vi "RichToFlatcif_can_writer_nixnet_Statistics.vi"(5 "OutputClusterType":T1, 11 "InputCluster":T2) -> (3 "OutputCluster":T1)   [LabVIEW 2021, in "CanWriterNixnet_server.lvlib"]
uses:
  CanWriterNixnet_server.lvlib
  cif_can_writer_nixnet_Statistics.ctl
  cif_can_writer_nixnet_Statistics_Flat.ctl
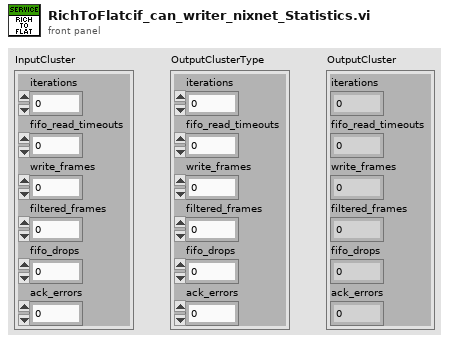
[diagram p1: front panel]
types:
  T1 = typedef "CanWriterNixnet_server.lvlib/cif_can_writer_nixnet_Statistics_Flat.ctl" = cluster{"iterations":u64, "fifo_read_timeouts":u64, "write_frames":u64, "filtered_frames":u64, "fifo_drops":u64, "ack_errors":u64}
  T2 = typedef "CanWriterNixnet_server.lvlib/cif_can_writer_nixnet_Statistics.ctl" = cluster{"iterations":u64, "fifo_read_timeouts":u64, "write_frames":u64, "filtered_frames":u64, "fifo_drops":u64, "ack_errors":u64}
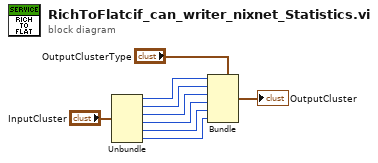
[diagram p0: block diagram]
diagram:
  n1 = Unbundle "Unbundle"("InputCluster") -> ("iterations"=w6:u64, "fifo_read_timeouts"=w5:u64, "write_frames"=w4:u64, "filtered_frames"=w3:u64, "fifo_drops"=w2:u64, "ack_errors"=w1:u64)
  n2 = Bundle "Bundle"(cluster="OutputClusterType", "iterations"=w6, "fifo_read_timeouts"=w5, "write_frames"=w4, "filtered_frames"=w3, "fifo_drops"=w2, "ack_errors"=w1) -> (→"OutputCluster":T1)
